vi "Start Periodic Enqueue Message.vi"(6 "Period [ms]":i32, 8 "error in (no error)":errorcluster, 9 "Message Data":variant, 10 "Message":string, 11 "MHL Queue":refnum<queue>) -> (0 "error out":errorcluster, 3 "Helper Loop":refnum<class "Helper Loop.lvclass">)   [LabVIEW 2024, in "Helper Loop.lvclass"]
doc: "入力したメッセージキュー、メッセージ、データ、周期で周期処理を開始します。\n無限待機中のヘルパーループが存在する場合はそのうちの1つを使用し、なければユーザーイベントを作成してヘルパーループを呼び出します。"
uses:
  Helper Loop.lvclass
  Helper Loop.lvclass/Helper Loop.ctl
  Sub/Helper Loop Core.vi
  support/Message Queue/Message Cluster.ctl
  support/Message Queue/Message Queue.lvlib
  Sub/Helper Loop Map FGV Action.ctl
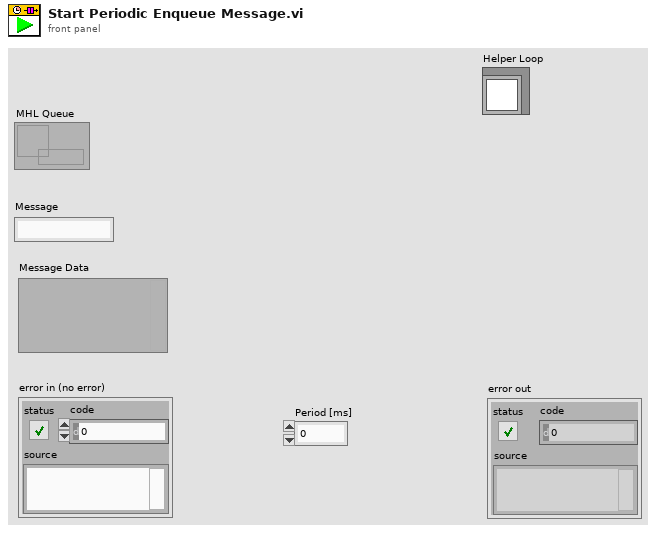
[diagram p1: front panel]
types:
  T1 = typedef "Helper Loop.lvclass/Helper Loop Map FGV Action.ctl" = enum16{"Get Pausing Helper Loop", "Register Active Helper Loop", "Pause Helper Loop", "Close Helper Loop", "Get All Helper Loops"}
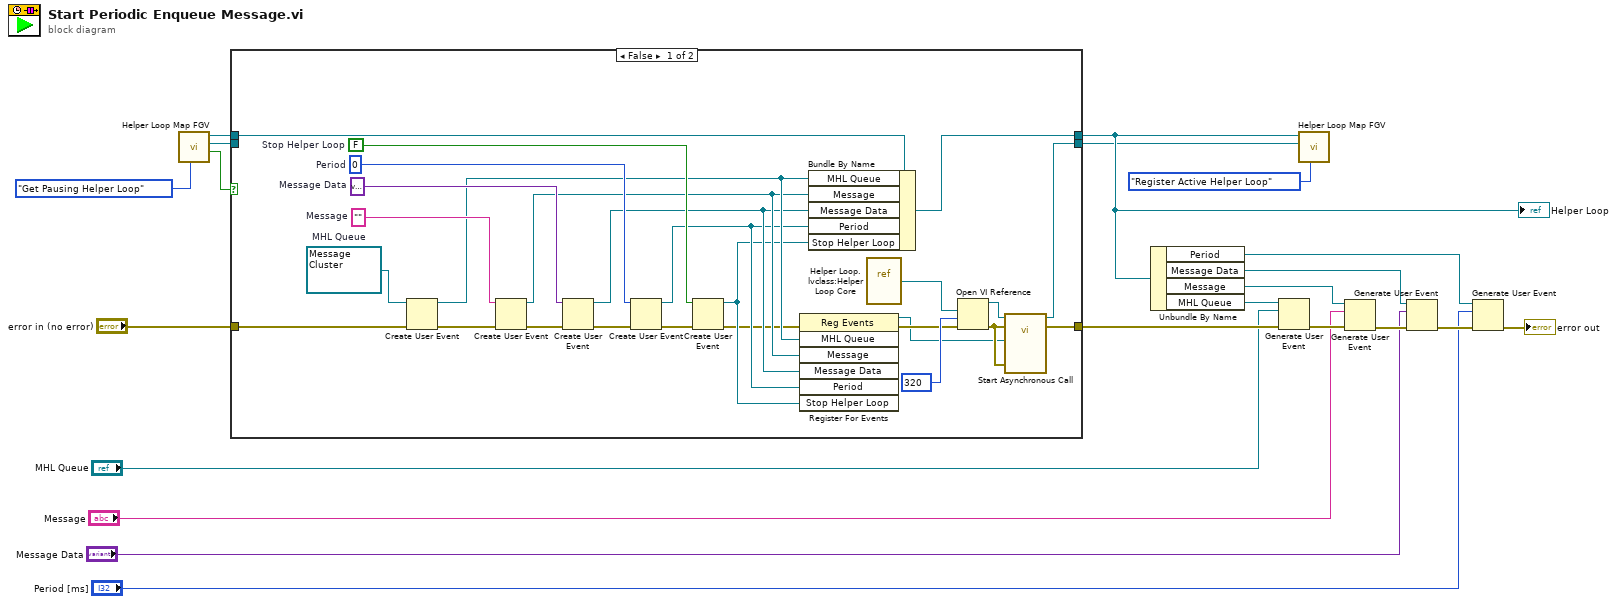
[diagram p0: block diagram]
diagram:
  n1 = call "Helper Loop Map FGV.vi"("Action"=Helper_Loop_Map_FGV_Action."Get Pausing Helper Loop") -> ("Get Helper Loop"=w6:bool, "Helper Loop VI Reference Out"=w2:refnum<vi>, "Helper Loop Out"=w5:refnum<class "Helper Loop.lvclass">)  [unwired: 7 in, 1 out]
  n2 = case shown="False" w6 {
    tunnel: "error in (no error)" -> [w34 w49]
    tunnel: [w33 w49] -> w20
    tunnel: [w31 w50] -> w3
    tunnel: w5 -> [w32 w50]
    tunnel: w2 -> [_ w48]
    tunnel: [w30 w48] -> w1
    frame False {
      w37 = FALSE  # Stop Helper Loop
      w42 = 0  # Period
      w43 = variant  # Message Data
      w44 = ""  # Message
      w45 = refnum<queue> refnum  # MHL Queue
      n3 = Create User Event(user event datatype=w45, error in=w34) -> (user event=w29:refnum<user-event>, error out=w41:errorcluster)
      n4 = Create User Event(user event datatype=w44, error in=w41) -> (user event=w28:refnum<user-event>, error out=w40:errorcluster)
      n5 = Create User Event(user event datatype=w43, error in=w40) -> (user event=w27:refnum<user-event>, error out=w39:errorcluster)
      n6 = Create User Event(user event datatype=w42, error in=w39) -> (user event=w26:refnum<user-event>, error out=w38:errorcluster)
      n7 = Create User Event(user event datatype=w37, error in=w38) -> (user event=w25:refnum<user-event>, error out=w24:errorcluster)
      n8 = register-events(error in=w24, w29, w28, w27, w26, w25) -> (reference out=w22:refnum<event-registration>, error out=w23:errorcluster)  [unwired: 1 in]
      n9 = Bundle By Name(cluster=w32, "MHL Queue"=w29, "Message"=w28, "Message Data"=w27, "Period"=w26, "Stop Helper Loop"=w25) -> (w31:refnum<class "Helper Loop.lvclass">)
      n10 = vi-ref "Helper Loop.lvclass:Helper Loop Core.vi"() -> (w46:refnum<vi>)
      n11 = Open VI Reference(vi path=w46, options=320, error in (no error)=w23) -> (vi reference=w36:refnum<vi>, error out=w35:errorcluster)  [unwired: 3 in]
      n12 = call-by-ref "Start Asynchronous Call"(reference=w36, error in=w35, "error in"=w35, "Event Registration Refnum"=w22) -> (reference out=w30:refnum<vi>, error out=w33:errorcluster)  [unwired: 9 in, 1 out]
    }
    frame True {
    }
  }
  "Helper Loop" <- w3
  n13 = Unbundle By Name(w3) -> ("Period"=w16:refnum<user-event>, "Message Data"=w15:refnum<user-event>, "Message"=w14:refnum<user-event>, "MHL Queue"=w13:refnum<user-event>)
  n14 = Generate User Event(user event=w13, event data cluster="MHL Queue", error in=w20) -> (error out=w19:errorcluster)  [unwired: 1 in, 1 out]
  n15 = call "Helper Loop Map FGV.vi"("Action"=Helper_Loop_Map_FGV_Action."Register Active Helper Loop", "Helper Loop VI Reference In"=w1, "Helper Loop In"=w3) -> ()  [unwired: 5 in, 4 out]
  n16 = Generate User Event(user event=w14, event data cluster="Message", error in=w19) -> (error out=w17:errorcluster)  [unwired: 1 in, 1 out]
  n17 = Generate User Event(user event=w15, event data cluster="Message Data", error in=w17) -> (error out=w18:errorcluster)  [unwired: 1 in, 1 out]
  n18 = Generate User Event(user event=w16, event data cluster="Period [ms]", error in=w18) -> (error out=→"error out":errorcluster)  [unwired: 1 in, 1 out]
